vi "Update CAN Status.vi"(8 "error in (no error)":errorcluster, 11 "XNET CAN RW in":refnum<class "XNET CAN RW.lvclass">) -> (0 "error out":errorcluster, 3 "XNET CAN RW out":refnum<class "XNET CAN RW.lvclass">)   [LabVIEW 2021, in "XNET CAN RW.lvclass"]
uses:
  XNET CAN RW.lvclass
  XNET CAN RW.lvclass/XNET CAN RW.ctl
  <vilib>/xnet/xnet.llb/XNET Read (State CAN Comm).vi
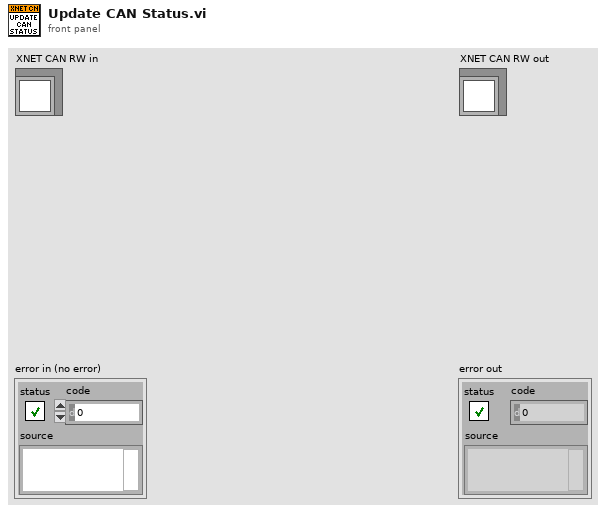
[diagram p1: front panel]
types:
  T1 = typedef "XNET CAN Comm.ctl" = cluster{"fault code":i32, "fault?":bool, "communication state":T2, "last error":T3, "receive error counter":u8, "transmit error counter":u8, "transceiver error?":bool, "sleep?":bool}
  T2 = typedef "XNET CAN Comm State.ctl" = u8
  T3 = typedef "XNET CAN Last Err.ctl" = u8
  T4 = typedef "CAN_RW_CORE.lvclass/CAN Status.ctl" = cluster{"Comm State":T5, "Last Error":T6, "RX Error Counter":u8, "TX Error Counter":u8}
  T5 = typedef "CAN_RW_CORE.lvclass/Communication State.ctl" = enum16{"Error Active", "Error Passive", "Bus Off"}
  T6 = typedef "CAN_RW_CORE.lvclass/Last Error.ctl" = enum16{"None", "Stuff", "Form", "Ack", "Bit1", "Bit0", "CRC", "Unknown"}
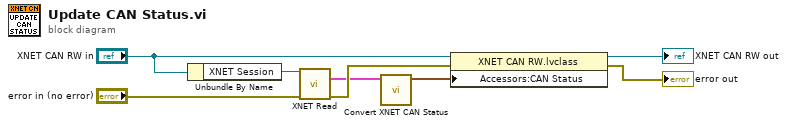
[diagram p0: block diagram]
diagram:
  n1 = Unbundle By Name("XNET CAN RW in") -> ("XNET Session"=w4:refnum<k21>)
  n2 = call-poly <vilib>:"XNET Read.vi"("session in"=w4, "error in (no error)"="error in (no error)") -> ("CAN comm"=w2:T1, "error out"=w3:errorcluster)  [unwired: 11 in, 1 out]
  n3 = call "Convert XNET CAN Status.vi"("CAN comm State"=w2) -> ("CAN Status"=w1:T4)  [unwired: 10 in]
  n4 = property class="XNET CAN RW.lvclass"(reference="XNET CAN RW in", error in=w3, "Accessors:CAN Status"=w1) -> (reference out=→"XNET CAN RW out":refnum<class "XNET CAN RW.lvclass">, error out=→"error out":errorcluster)
